vi "Export Groups.vi"(8 "error in (no error)":errorcluster, 10 "Path":path, 11 "BluelinesRedlines in":refnum<class "BluelinesRedlines.lvclass">) -> (0 "error out":errorcluster, 3 "BluelinesRedlines out":refnum<class "BluelinesRedlines.lvclass">)   [LabVIEW 2020, in "VolatusGUIElements.lvlib" / "BluelinesRedlines.lvclass"]
uses:
  BluelinesRedlines.lvclass
  BluelinesRedlines.lvclass/BluelinesRedlines.ctl
  User BluelinesRedlines/User BluelinesRedlines.lvclass
  lv-cdm/CDM-Config/Config-JSON/Config-JSON.lvclass
  C:/dev/lv20CE/relink/lv-cdm/CDM-Config/Config Storage/Config Storage.lvclass
  lv-cdm/CDM-Config/Config Element/Write Variant Value.vi
  lv-cdm/CDM-Config/Config Manager/Config Manager.lvclass
  lv-cdm/CDM-Config/Config Element/Config Element.lvclass
  lv-cdm/CDM-Config/Config Storage/Config Storage.lvclass
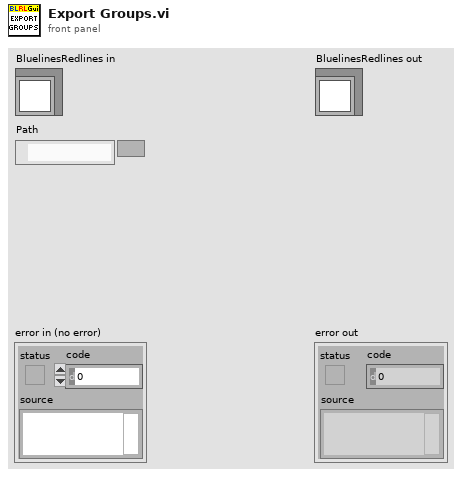
[diagram p1: front panel]
types:
  T1 = map{string, refnum<class "BluelinesRedlines Source.lvclass">}
  T2 = typedef "VolatusGUI.lvlib/BluelinesRedlines Source.lvclass/BLRL Config.ctl" = cluster{"Bluelines":T3[], "Redlines":T3[]}
  T3 = typedef "VolatusGUI.lvlib/BluelinesRedlines Source.lvclass/Range Limit Config.ctl" = cluster{"Channel":string, "Low Limit":dbl, "High Limit":dbl}
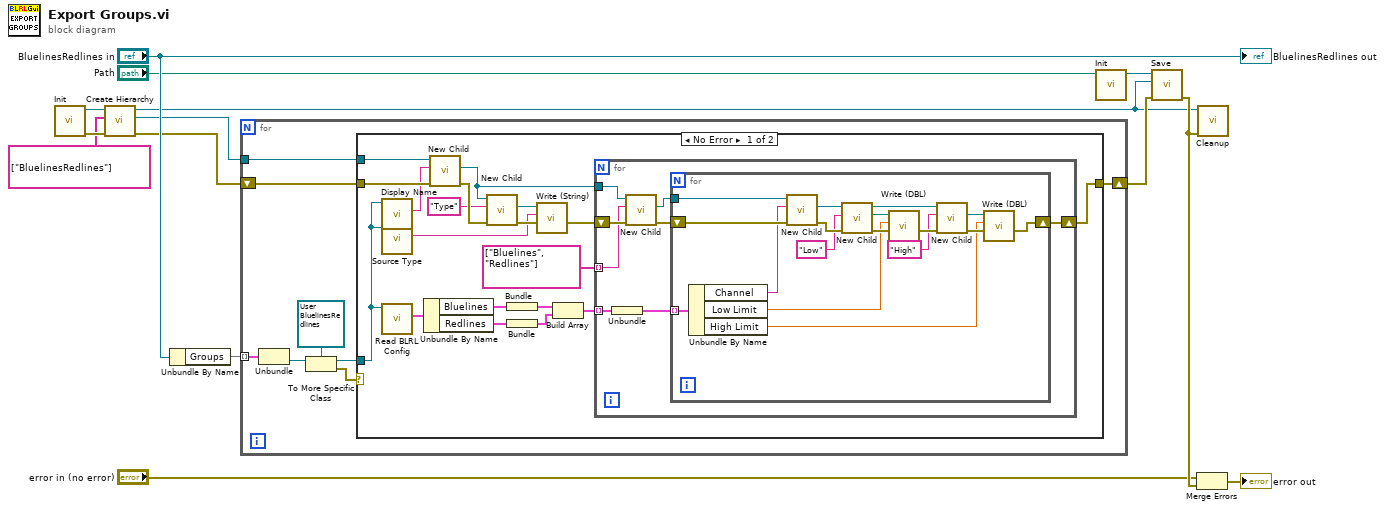
[diagram p0: block diagram]
diagram:
  n1 = call "Init.vi"() -> ("error out"=w11:errorcluster, "Config Manager out"=w10:refnum<class "Config Manager.lvclass">)  [unwired: 10 in]
  n2 = call "Create Hierarchy.vi"("error in (no error)"=w11, "Hierarchy"=string[] ["BluelinesRedlines"], "Config Manager in"=w10) -> ("error out"=w8:errorcluster, "Leaf Element"=w7:refnum<class "Config Element.lvclass">, "Config Manager out"=w1:refnum<class "Config Manager.lvclass">)  [unwired: 6 in]
  n3 = Unbundle By Name("BluelinesRedlines in") -> ("Groups"=w12:T1)
  n4 = for {
    tunnel: w12 -> [w22] mode=indexing
    shift-right: [w15] -> w4
    shift-left: w8 -> [w16]
    tunnel: w7 -> [w17]
    n5 = Unbundle(w22) -> ("VolatusGUI:BluelinesRedlines Source.lvclass"=w21:refnum<class "BluelinesRedlines Source.lvclass">)  [unwired: 1 out]
    n6 = To More Specific Class(target class=refnum<class "User BluelinesRedlines.lvclass"> refnum ("VolatusGUIElements.lvlib:User BluelinesRedlines.lvclass"), reference=w21) -> (specific class reference=w18:refnum<class "User BluelinesRedlines.lvclass">, error out=w19:errorcluster)  [unwired: 1 in]
    n7 = case shown="No Error" w19 {
      tunnel: w18 -> [w33 _]
      tunnel: w17 -> [w41 _]
      tunnel: w16 -> [w40 w67]
      tunnel: [w23 w67] -> w15
      frame No Error {
        n8 = call-dynamic "Display Name.vi"("User BluelinesRedlines in"=w33) -> ("Display Name"=w39:string)  [unwired: 10 in]
        n9 = call-dynamic "Source Type.vi"("User BluelinesRedlines in"=w33) -> ("Source Type"=w34:string)  [unwired: 10 in]
        n10 = call-dynamic "Read BLRL Config.vi"("User BluelinesRedlines in"=w33) -> ("BLRL Config"=w32:T2)  [unwired: 8 in, 2 out]
        n11 = Unbundle By Name(w32) -> ("Bluelines"=w31:T3[], "Redlines"=w30:T3[])
        n12 = call "New Child.vi"("error in (no error)"=w40, "Child Name"=w39, "Config Element in"=w41) -> ("error out"=w38:errorcluster, "New Child"=w26:refnum<class "Config Element.lvclass">)  [unwired: 6 in, 1 out]
        n13 = call "New Child.vi"("error in (no error)"=w38, "Child Name"="Type", "Config Element in"=w26) -> ("error out"=w36:errorcluster, "New Child"=w35:refnum<class "Config Element.lvclass">)  [unwired: 6 in, 1 out]
        n14 = Bundle("Bluelines"=w31) -> (w29:cluster{"Bluelines":T3[]})  [unwired: 1 in]
        n15 = Bundle("Redlines"=w30) -> (w28:cluster{"Redlines":T3[]})  [unwired: 1 in]
        n16 = call "Write (String).vi"("error in (no error)"=w36, "String Value"=w34, "Config Element in"=w35) -> ("error out"=w25:errorcluster)  [unwired: 7 in, 1 out]
        n17 = Build Array(w29, w28) -> (w27:cluster{"Redlines":T3[]}[])
        n18 = for {
          tunnel: w27 -> [w46] mode=indexing
          tunnel: w26 -> [w48]
          shift-right: [w42] -> w23
          shift-left: w25 -> [w49]
          tunnel: string[] ["Bluelines", "Redlines"] -> [w47] mode=indexing
          n19 = Unbundle(w46) -> ("Redlines"=w43:T3[])
          n20 = call "New Child.vi"("error in (no error)"=w49, "Child Name"=w47, "Config Element in"=w48) -> ("error out"=w45:errorcluster, "New Child"=w44:refnum<class "Config Element.lvclass">)  [unwired: 6 in, 1 out]
          n21 = for {
            shift-right: [w50] -> w42
            shift-left: w45 -> [w66]
            tunnel: w44 -> [w65]
            tunnel: w43 -> [w64] mode=indexing
            n22 = Unbundle By Name(w64) -> ("Channel"=w63:string, "Low Limit"=w57:dbl, "High Limit"=w51:dbl)
            n23 = call "New Child.vi"("error in (no error)"=w66, "Child Name"=w63, "Config Element in"=w65) -> ("error out"=w61:errorcluster, "New Child"=w62:refnum<class "Config Element.lvclass">)  [unwired: 6 in, 1 out]
            n24 = call "New Child.vi"("error in (no error)"=w61, "Child Name"="Low", "Config Element in"=w62) -> ("error out"=w59:errorcluster, "New Child"=w58:refnum<class "Config Element.lvclass">, "Config Element out"=w53:refnum<class "Config Element.lvclass">)  [unwired: 6 in]
            n25 = call "Write (DBL).vi"("error in (no error)"=w59, "DBL Value"=w57, "Config Element in"=w58) -> ("error out"=w54:errorcluster)  [unwired: 7 in, 1 out]
            n26 = call "New Child.vi"("error in (no error)"=w54, "Child Name"="High", "Config Element in"=w53) -> ("error out"=w55:errorcluster, "New Child"=w56:refnum<class "Config Element.lvclass">)  [unwired: 6 in, 1 out]
            n27 = call "Write (DBL).vi"("error in (no error)"=w55, "DBL Value"=w51, "Config Element in"=w56) -> ("error out"=w50:errorcluster)  [unwired: 7 in, 1 out]
          }
        }
      }
      frame Error {
        # "Not a User defined group, do not export."
      }
    }
  }
  n28 = call "Init.vi"("Path"="Path") -> ("Config-JSON out"=w5:refnum<class "Config-JSON.lvclass">)  [unwired: 9 in, 1 out]
  n29 = call "Save.vi"("error in (no error)"=w4, "Config"=w1, "Config Storage in"=w5) -> ("error out"=w14:errorcluster)  [unwired: 7 in, 1 out]
  n30 = Merge Errors("error in (no error)", w14) -> (→"error out":errorcluster)
  n31 = call "Cleanup.vi"("error in (no error)"=w14, "Config Manager in"=w1) -> ()  [unwired: 9 in, 1 out]
  "BluelinesRedlines out" <- "BluelinesRedlines in"
